vi "Read_Diagnostics.vi"(8 "error in (no error)":errorcluster, 11 "WEG_SCA06_Modbus in":refnum<class "WEG_SCA06_Modbus.lvclass">) -> (0 "error out":errorcluster, 2 "Diagnostics":T1, 3 "WEG_SCA06_Modbus out":refnum<class "WEG_SCA06_Modbus.lvclass">)   [LabVIEW 2021, in "WEG_SCA06_Modbus.lvclass"]
uses:
  WEG_SCA06_Modbus.lvclass
  WEG_SCA06_Modbus.lvclass/WEG_SCA06_Modbus.ctl
  Modbus_Master/Modbus_Master.lvclass
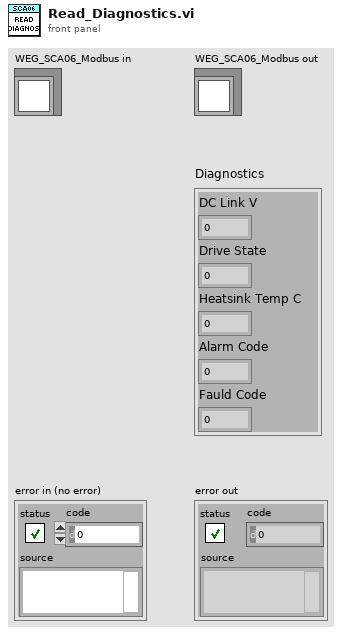
[diagram p1: front panel]
types:
  T1 = cluster{"DC Link V":dbl, "Drive State":u16, "Heatsink Temp C":dbl, "Alarm Code":dbl, "Fauld Code":dbl}
  T2 = cluster{"register":u16, "register":u16, "register":u16, "register":u16, "register":u16}
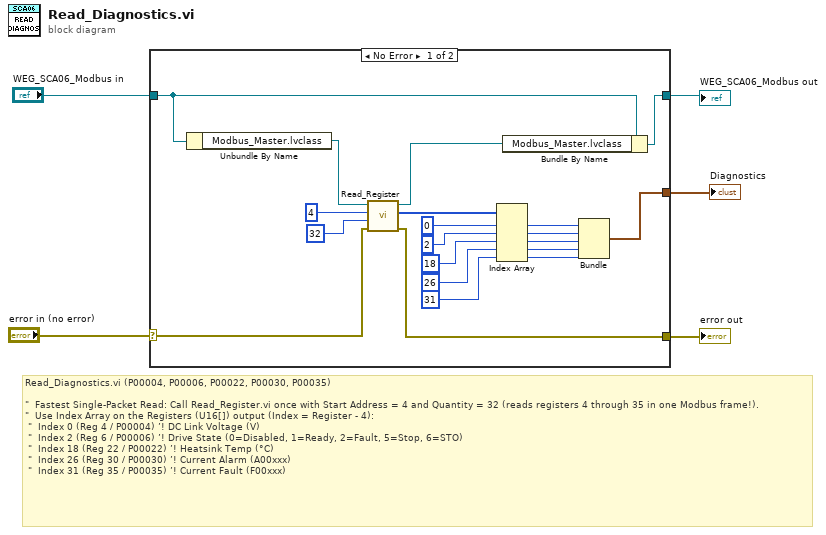
[diagram p0: block diagram]
diagram:
  # "Read_Diagnostics.vi (P00004, P00006, P00022, P00030, P00035)\n\n\"  Fastest Single-Packet Read: Call Read_Register.vi once with Start Address = 4 and Quantity = 32 (reads registers 4 through 35 in one Modbus frame!).\n\"  Use Index Array on the Registers (U16[]) output (Index = Register - 4):\n\t\"  Index 0 (Reg 4 / P00004) ’! DC Link Voltage (V)\n\t\"  Index 2 (Reg 6 / P00006) ’! Drive State (0=Disabled, 1=Ready, 2=Fault, 5=Stop, 6=STO)\n\t\"  Index 18 (Reg 22 / P00022) ’! Heatsink Temp (°C)\n\t\"  Index 26 (Reg 30 / P00030) ’! Current Alarm (A00xxx)\n\t\"  Index 31 (Reg 35 / P00035) ’! Current Fault (F00xxx)"
  n1 = case shown="No Error" "error in (no error)" {
    selector: "error in (no error)" -> [w20 w27]
    tunnel: [w18 w27] -> w4
    tunnel: "WEG_SCA06_Modbus in" -> [w25 w26]
    tunnel: [w24 w26] -> w2
    tunnel: [w6 _] -> w1
    frame No Error {
      n2 = Unbundle By Name(w25) -> ("Modbus_Master.lvclass"=w23:refnum<class "Modbus_Master.lvclass">)
      n3 = call "Read_Register.vi"("error in (no error)"=w20, "Quantity"=u16 32, "Start Address"=u16 4, "Modbus_Master in"=w23) -> ("error out"=w18:errorcluster, "register values"=w17:u16[], "Modbus_Master out"=w19:refnum<class "Modbus_Master.lvclass">)  [unwired: 5 in]
      n4 = Index Array(array=w17, index #1=0 ("index"), index #2=2 ("index"), index #3=18 ("index"), index #4=26 ("index"), index #5=31 ("index")) -> (element #1=w11:u16, element #2=w10:u16, element #3=w9:u16, element #4=w8:u16, element #5=w7:u16)
      n5 = Bundle By Name(cluster=w25, "Modbus_Master.lvclass"=w19) -> (w24:refnum<class "WEG_SCA06_Modbus.lvclass">)
      n6 = Bundle("register"=w11, "register"=w10, "register"=w9, "register"=w8, "register"=w7) -> (w6:T2)  [unwired: 1 in]
    }
    frame Error {
    }
  }
  "error out" <- w4
  "WEG_SCA06_Modbus out" <- w2
  "Diagnostics" <- w1
